vi "VIH Project - Verify CSS,JS,Template Files - Group Rule.vi"(10 "Group Rule":T1, 11 "Group name":string) -> (2 "Bad files":path[](array[path]))   [LabVIEW 2014]
doc: "::: VI Helpeks :::\nCopyright (c) 2000-2026 Konstantin Shifershteyn. All rights reserved."
uses:
  _VIH HelpGen.llb/VIH HelpGen Typedef - Cluster - Group Rule.ctl
  _VIH HelpGen.llb/VIH HelpGen Typedef - Enum - Default,Enable,Disable.ctl
  _VIH HelpGen.llb/VIH HelpGen Typedef - Cluster - Group Rule - Source Paths.ctl
  _VIH HelpGen.llb/VIH HelpGen Typedef - Cluster - Group Rule - Target Paths.ctl
  _VIH HelpGen.llb/VIH HelpGen Typedef - Enum - Description Mode.ctl
  _VIH HelpGen.llb/VIH HelpGen Typedef - Cluster - Control Rule.ctl
  _VIH HelpGen.llb/VIH HelpGen Typedef - Cluster - Enum Value Info.ctl
  _VIH HelpGen.llb/VIH HelpGen Typedef - Cluster - Group Rule - Flags.ctl
panel:
  # "VI Helpeks\nCopyright (c) 2012-2026 Konstantin Shifershteyn"
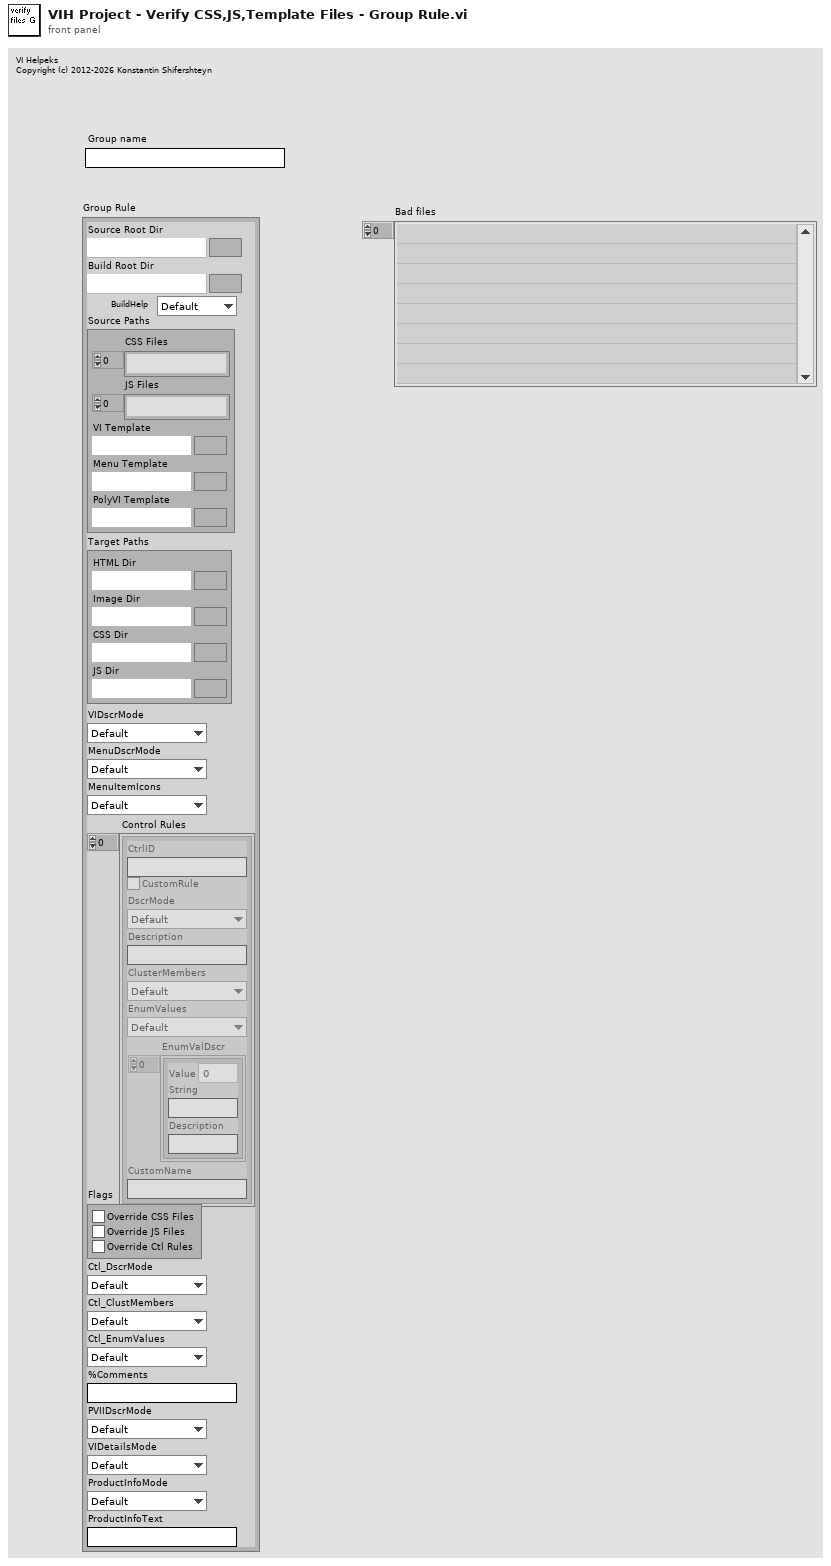
[diagram p1: front panel]
types:
  T1 = typedef "VIH HelpGen Typedef - Cluster - Group Rule.ctl" = cluster{"Source Root Dir":path, "Build Root Dir":path, "BuildHelp":T2, "Source Paths":T3, "Target Paths":T4, "VIDscrMode":T5, "MenuDscrMode":T5, "MenuItemIcons":T2, "Control Rules":T6[], "Flags":T8, "Ctl_DscrMode":T5, "Ctl_ClustMembers":T2, "Ctl_EnumValues":T2, "%Comments":string, "PVIIDscrMode":T5, "VIDetailsMode":T5, "ProductInfoMode":T2, "ProductInfoText":string}
  T2 = typedef "VIH HelpGen Typedef - Enum - Default,Enable,Disable.ctl" = enum16{"Default", "Enable", "Disable"}
  T3 = typedef "VIH HelpGen Typedef - Cluster - Group Rule - Source Paths.ctl" = cluster{"CSS Files":path[], "JS Files":path[], "VI Template":path, "Menu Template":path, "PolyVI Template":path}
  T4 = typedef "VIH HelpGen Typedef - Cluster - Group Rule - Target Paths.ctl" = cluster{"HTML Dir":path, "Image Dir":path, "CSS Dir":path, "JS Dir":path}
  T5 = typedef "VIH HelpGen Typedef - Enum - Description Mode.ctl" = enum16{"Default", "Description", "Description1", "Description2", "Custom", "None"}
  T6 = typedef "VIH HelpGen Typedef - Cluster - Control Rule.ctl" = cluster{"CtrlID":string, "CustomRule":bool, "DscrMode":T5, "Description":string, "ClusterMembers":T2, "EnumValues":T2, "EnumValDscr":T7[], "CustomName":string}
  T7 = typedef "VIH HelpGen Typedef - Cluster - Enum Value Info.ctl" = cluster{"Value":ext, "String":string, "Description":string}
  T8 = typedef "VIH HelpGen Typedef - Cluster - Group Rule - Flags.ctl" = cluster{"Override CSS Files":bool, "Override JS Files":bool, "Override Ctl Rules":bool}
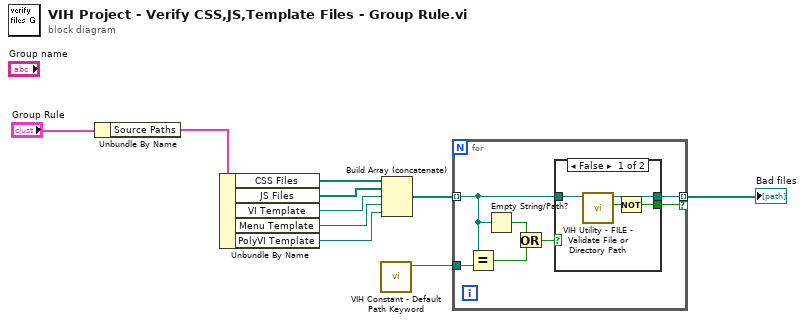
[diagram p0: block diagram]
diagram:
  n1 = Unbundle By Name("Group Rule") -> ("Source Paths"=w9:T3)
  n2 = Unbundle By Name(w9) -> ("CSS Files"=w8:path[], "JS Files"=w7:path[], "VI Template"=w6:path, "Menu Template"=w5:path, "PolyVI Template"=w4:path)
  n3 = call "VIH Constant - Default Path Keyword.vi"() -> ("<default> path"=w1:path)  [unwired: 11 in]
  n4 = Build Array (concatenate)(w8, w7, w6, w5, w4) -> (w3:path[])
  n5 = for {
    tunnel: w3 -> [w14] mode=indexing
    tunnel: w1 -> [w17]
    tunnel: [w13] -> w2 mode=indexing if=w11
    n6 = Equal?(x=w14, y=w17) -> (x = y?=w15:bool)
    n7 = Empty String/Path?(string/path=w14) -> (empty?=w16:bool)
    n8 = Or(x=w16, y=w15) -> (x .or. y?=w12:bool)
    n9 = case shown="False" w12 {
      tunnel: w14 -> [w21 w22]
      tunnel: [w20 w22] -> w13
      tunnel: [w18 _] -> w11
      frame False {
        n10 = call "VIH Utility - FILE - Validate File or Directory Path.vi"("Path"=w21) -> ("file"=w19:bool, "dup Path"=w20:path)  [unwired: 6 in, 3 out]
        n11 = Not(x=w19) -> (.not. x?=w18:bool)
      }
      frame True {
      }
    }
  }
  "Bad files" <- w2
